vi "Get Feature Representation.vi"(8 "error in (no error)":errorcluster, 10 "Feature":string, 11 "Camera in":refnum<class "Camera.lvclass">) -> (0 "error out":errorcluster, 2 "Representation":T1, 3 "Camera":refnum<class "Camera.lvclass">)   [LabVIEW 2020, in "Camera.lvclass"]
uses:
  Camera.lvclass
  Representation.ctl
  Camera.lvclass/Camera.ctl
  bin/gindustrialcam_32-1.dll
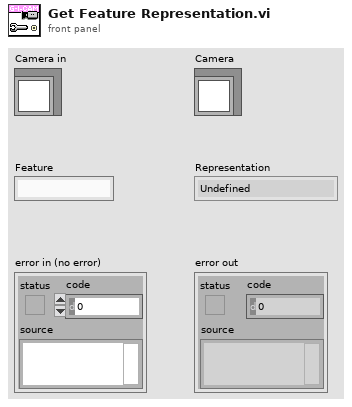
[diagram p1: front panel]
types:
  T1 = typedef "Camera.lvclass/Representation.ctl" = enum8{"Undefined", "Linear", "Logarithmic", "Boolean", "Pure Number", "Hex Number", "IP Address", "MAC Address"}
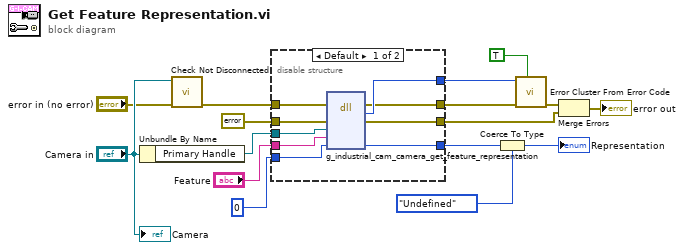
[diagram p0: block diagram]
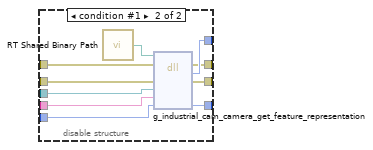
[diagram p2: hidden frame]
diagram:
  n1 = Unbundle By Name("Camera in") -> ("Primary Handle"=w12:refnum<data-value>)
  n2 = call "Check Not Disconnected.vi"("error in (no error)"="error in (no error)", "Camera in"="Camera in") -> ("error out"=w13:errorcluster)  [unwired: 9 in]
  n3 = disable-structure shown="Default" {
    disable-tunnel: w13 -> [w25 w35]
    disable-tunnel: w12 -> [w24 w34]
    disable-tunnel: errorcluster {"status"=FALSE, "code"=0, "source"=""} ("error constant") -> [w23 w33]
    disable-tunnel: [w22 w32] -> w9
    disable-tunnel: [w21 w31] -> w7
    disable-tunnel: [w20 w30] -> w6
    disable-tunnel: "Feature" -> [w19 w29]
    disable-tunnel: [w18 w28] -> w3
    disable-tunnel: u8 0 ("representation") -> [w17 w27]
    frame condition #0 (active) {
      n4 = dll-call lib="C:/serenial/lib/g-industrial-camera/LabVIEW/g_industrial_cam/bin/gindustrialcam_*-1.*" fn="g_industrial_cam_camera_get_feature_representation"(error in=w25, "err"=w23, "edvr"=w24, "feature"=w19, "representation"=w17) -> (error out=w20:errorcluster, "Mg_Error"=w21:i32, "err"=w22:errorcluster, "representation"=w18:u8)  [unwired: 4 in, 1 out]
    }
    frame condition #1 {
      n5 = call "RT Shared Binary Path.vi"() -> ("Path"=w26:path)
      n6 = dll-call lib="C:/serenial/lib/g-industrial-camera/LabVIEW/g_industrial_cam/bin/gindustrialcam_*-1.*" fn="g_industrial_cam_camera_get_feature_representation"(path in=w26, error in=w35, "err"=w33, "edvr"=w34, "feature"=w29, "representation"=w27) -> (error out=w30:errorcluster, "Mg_Error"=w31:i32, "err"=w32:errorcluster, "representation"=w28:u8)  [unwired: 3 in, 1 out]
    }
  }
  n7 = Coerce To Type(0:w3, 1:Representation."Undefined" ("Representation")) -> (2:→"Representation":T1)
  n8 = call <vilib>:"Error Cluster From Error Code.vi"("show call chain? (False)"=TRUE, "error in (no error)"=w6, "error code (0)"=w7) -> ("error out"=w8:errorcluster)  [unwired: 6 in]
  n9 = Merge Errors(w8, w9) -> (→"error out":errorcluster)
  "Camera" <- "Camera in"
